vi "RemoteVI Hide Window.vi"(0 "hwnd":u64, 11 "error in":errorcluster) -> (4 "hidden?":bool, 15 "error out":errorcluster)   [LabVIEW 2020, in "RemoteVI.lvlib"]
doc: "Makes the top-level window hwnd invisible on the host screen while it stays open and functional: adds the extended style WS_EX_LAYERED (0x80000) with SetWindowLongPtrW(GWL_EXSTYLE -20) unless it is already set, then sets the opacity to 0 with SetLayeredWindowAttributes(alpha 0, LWA_ALPHA 2). Used for LabVIEW popups (menus, drop-downs, graph palette popups and their SysShadow) that a REMOTE user opened, so they do not float over the host's desktop; RemoteVI Capture Window.vi still captures them and posted clicks still reach them (measured). Idempotent. Win32 only, no VI Server call."
uses:
  RemoteVI.lvlib
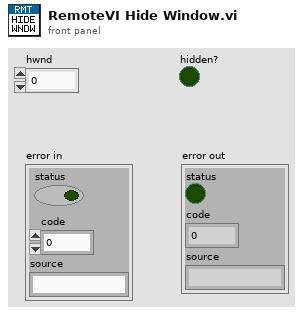
[diagram p1: front panel]
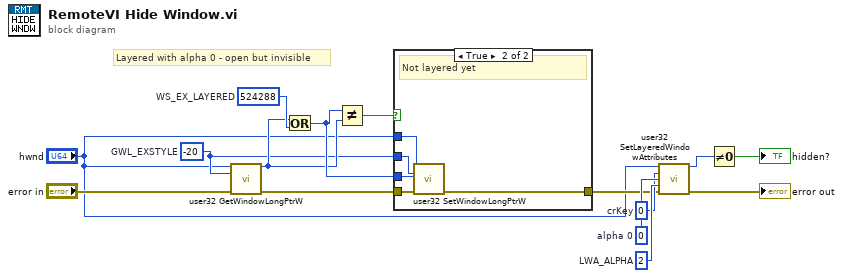
[diagram p0: block diagram]
diagram:
  w14 = u32 2  # LWA_ALPHA
  w13 = u8 0  # alpha 0
  w12 = u32 0  # crKey
  w8 = i64 524288  # WS_EX_LAYERED
  w5 = -20  # GWL_EXSTYLE
  # "Layered with alpha 0 - open but invisible"
  n1 = call "user32 GetWindowLongPtrW.vi"("hWnd"="hwnd", "nIndex"=w5, "error in"="error in") -> ("return value"=w6:i64, "error out"=w7:errorcluster)  [unwired: 11 in]
  n2 = Or(x=w6, y=w8) -> (x .or. y?=w9:i64)
  n3 = Not Equal?(x=w9, y=w6) -> (x != y?=w10:bool)
  n4 = case shown="True" w10 {
    tunnel: "hwnd" -> [_ w17]
    tunnel: w5 -> [_ w18]
    tunnel: w7 -> [w16 w20]
    tunnel: w9 -> [_ w19]
    tunnel: [w16 w21] -> w11
    frame False {
      # "Already layered"
    }
    frame True {
      # "Not layered yet"
      n5 = call "user32 SetWindowLongPtrW.vi"("hWnd"=w17, "nIndex"=w18, "dwNewLong"=w19, "error in"=w20) -> ("error out"=w21:errorcluster)  [unwired: 10 in, 1 out]
    }
  }
  n6 = call "user32 SetLayeredWindowAttributes.vi"("hwnd"="hwnd", "crKey"=w12, "bAlpha"=w13, "dwFlags"=w14, "error in"=w11) -> ("return value"=w15:i32, "error out"=→"error out":errorcluster)  [unwired: 9 in]
  n7 = Not Equal To 0?(x=w15) -> (x != 0?=→"hidden?":bool)
